vi "Matrix_Pow.vi"(10 "Exponent":dbl, 11 "input matrix":T1) -> (0 "Error":bool, 3 "output matrix":T1, 4 "ExponentNotRational":bool)   [LabVIEW 2019, in "Trajectory_Library.lvlib"]
doc: "Computes the matrix power using Eigen's solver. This method only works for square matrices, and will otherwise throw an MatrixDimensionException.\n \nInputs:\n - input matrix -- The input matrix\n - exponent -- The exponent.\n\nOutputs:\n - output matrix -- The exponential of A.\n - error -- If TRUE, an error occured.\n - ExponentNotRational -- TRUE if exponent is not a rational number."
uses:
  Trajectory_Library.lvlib
  <vilib>/Analysis/Matrix/Datatypes/RealMatrix.ctl
  <vilib>/Analysis/7linalg.llb/Real Matrix Power.vi
  <vilib>/Analysis/7linalg.llb/Real Matrix Exp.vi
  <vilib>/Analysis/7linalg.llb/Real Matrix Logarithm.vi
  <vilib>/Analysis/Matrix/Numeric/Complex/Complex To Cartesian - CM.vi
  <vilib>/Analysis/Matrix/Numeric/Multiply/Multiply - RM,R.vi
  <vilib>/Analysis/NI_AALBase.lvlib
  <vilib>/Analysis/Matrix/NI_Matrix.lvlib
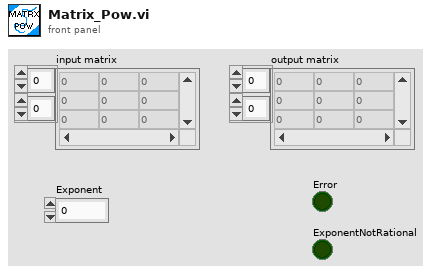
[diagram p1: front panel]
types:
  T1 = typedef "NI_Matrix.lvlib/RealMatrix.ctl" = dbl[][]
  T2 = typedef "NI_Matrix.lvlib/ComplexMatrix.ctl" = cdb[][]
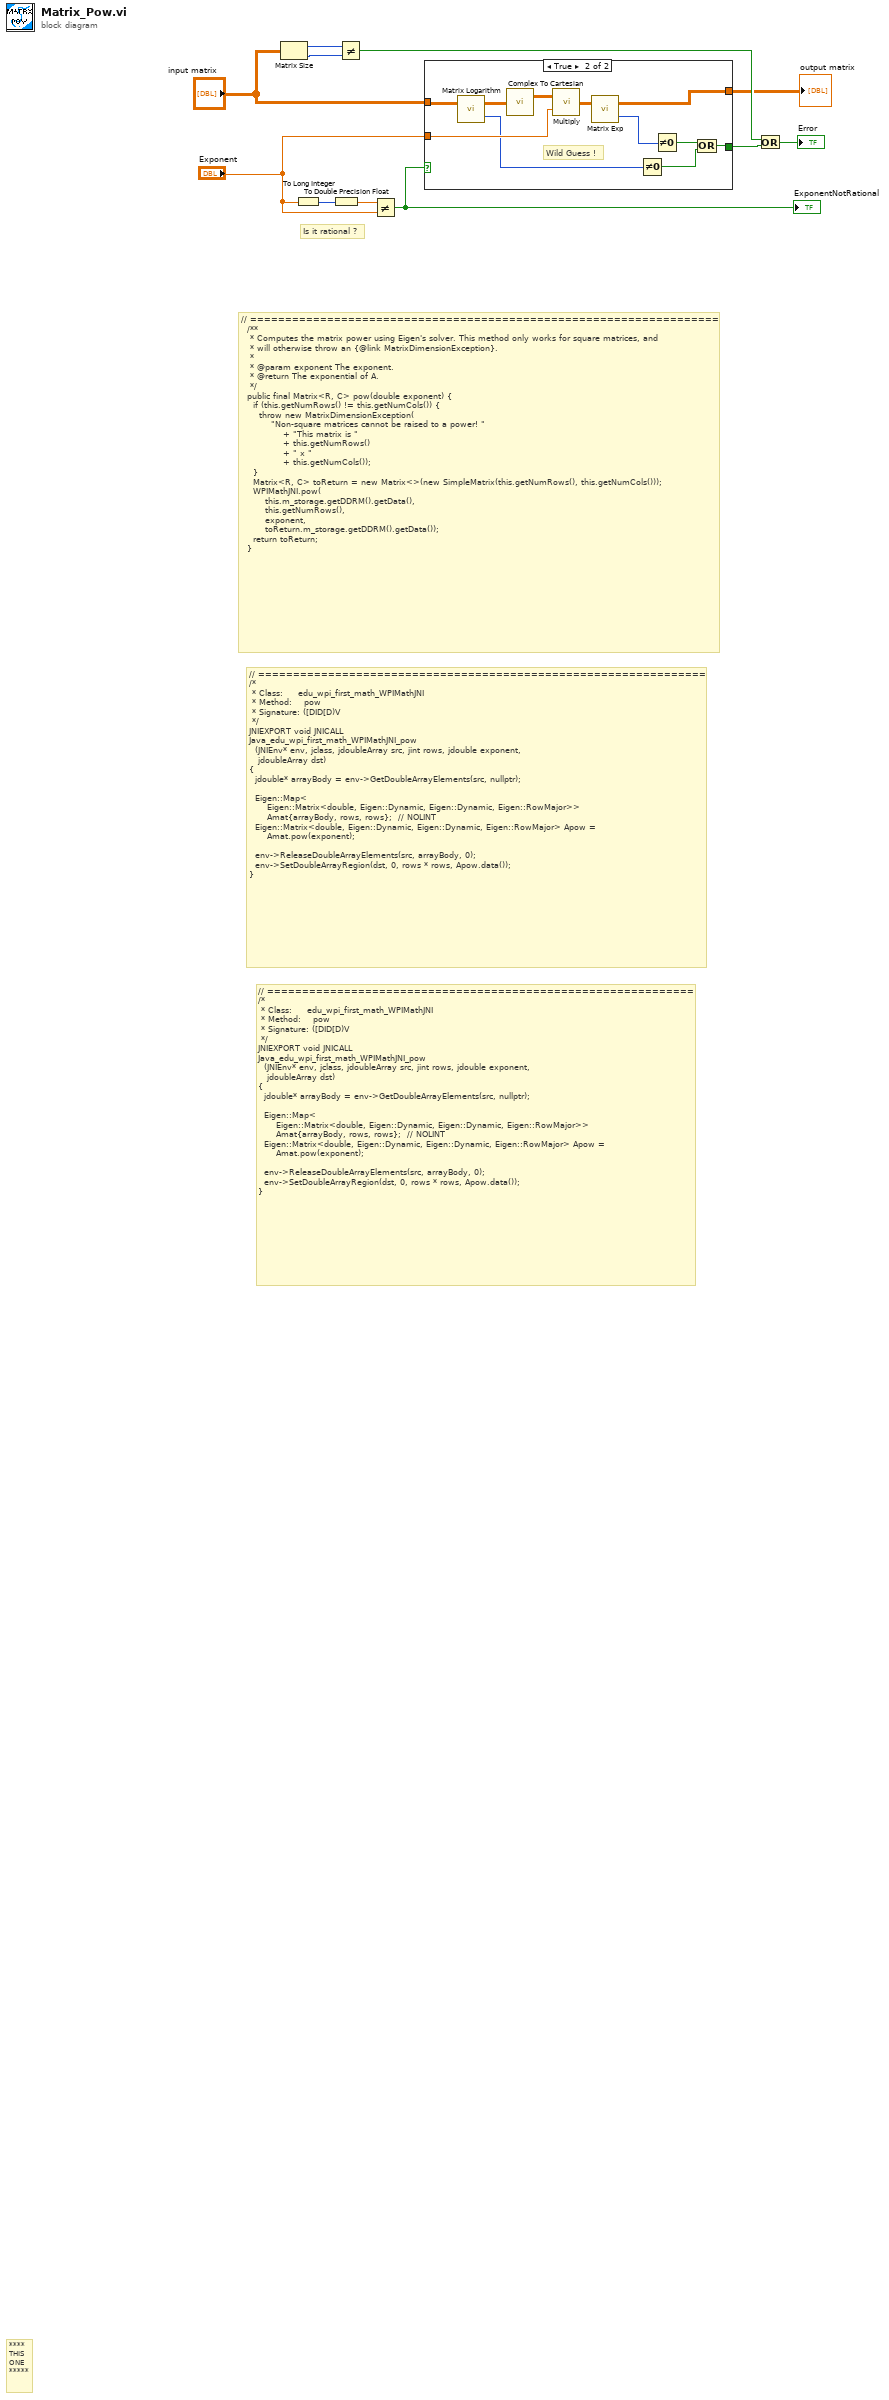
[diagram p0: block diagram]
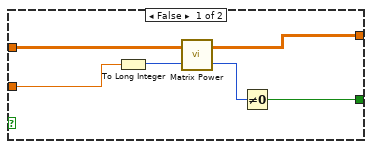
[diagram p2: hidden frame]
diagram:
  # "Is it rational ?"
  # "// =============================================================\n/*\n * Class:     edu_wpi_first_math_WPIMathJNI\n * Method:    pow\n * Signature: ([DID[D)V\n */\nJNIEXPORT void JNICALL\nJava_edu_wpi_first_math_WPIMathJNI_pow\n  (JNIEnv* env, jclass, jdoubleArray src, jint rows, jdouble exponent,\n   jdoubleArray dst)\n{\n  jdouble* arrayBody = env->GetDoubleArrayElements(src, nullptr);\n\n  Eigen::Map<\n      Eigen::Matrix<double, Eigen::Dynamic, Eigen::Dynamic, Eigen::RowMajor>>\n      Amat{arrayBody, rows, rows};  // NOLINT\n  Eigen::Matrix<double, Eigen::Dynamic, Eigen::Dynamic, Eigen::RowMajor> Apow =\n      Amat.pow(exponent);\n\n  env->ReleaseDoubleArrayElements(src, arrayBody, 0);\n  env->SetDoubleArrayRegion(dst, 0, rows * rows, Apow.data());\n}"
  # "// ================================================================\n/*\n * Class:     edu_wpi_first_math_WPIMathJNI\n * Method:    pow\n * Signature: ([DID[D)V\n */\nJNIEXPORT void JNICALL\nJava_edu_wpi_first_math_WPIMathJNI_pow\n  (JNIEnv* env, jclass, jdoubleArray src, jint rows, jdouble exponent,\n   jdoubleArray dst)\n{\n  jdouble* arrayBody = env->GetDoubleArrayElements(src, nullptr);\n\n  Eigen::Map<\n      Eigen::Matrix<double, Eigen::Dynamic, Eigen::Dynamic, Eigen::RowMajor>>\n      Amat{arrayBody, rows, rows};  // NOLINT\n  Eigen::Matrix<double, Eigen::Dynamic, Eigen::Dynamic, Eigen::RowMajor> Apow =\n      Amat.pow(exponent);\n\n  env->ReleaseDoubleArrayElements(src, arrayBody, 0);\n  env->SetDoubleArrayRegion(dst, 0, rows * rows, Apow.data());\n}"
  # "// ===================================================================\n  /**\n   * Computes the matrix power using Eigen's solver. This method only works for square matrices, and\n   * will otherwise throw an {@link MatrixDimensionException}.\n   *\n   * @param exponent The exponent.\n   * @return The exponential of A.\n   */\n  public final Matrix<R, C> pow(double exponent) {\n    if (this.getNumRows() != this.getNumCols()) {\n      throw new MatrixDimensionException(\n          \"Non-square matrices cannot be raised to a power! \"\n              + \"This matrix is \"\n              + this.getNumRows()\n              + \" x \"\n              + this.getNumCols());\n    }\n    Matrix<R, C> toReturn = new Matrix<>(new SimpleMatrix(this.getNumRows(), this.getNumCols()));\n    WPIMathJNI.pow(\n        this.m_storage.getDDRM().getData(),\n        this.getNumRows(),\n        exponent,\n        toReturn.m_storage.getDDRM().getData());\n    return toReturn;\n  }"
  # "****\nTHIS\nONE\n*****"
  n1 = Matrix Size(0:"input matrix") -> (1:w11:i32, 2:w10:i32)
  n2 = To Long Integer(number="Exponent") -> (32bit integer=w7:i32)
  n3 = To Double Precision Float(number=w7) -> (double precision float=w6:dbl)
  n4 = Not Equal?(x=w11, y=w10) -> (x != y?=w8:bool)
  n5 = Not Equal?(x=w6, y="Exponent") -> (x != y?=w5:bool)
  "ExponentNotRational" <- w5
  n6 = case shown="True" w5 {
    tunnel: "input matrix" -> [w17 w28]
    tunnel: "Exponent" -> [w12 w27]
    tunnel: [w15 w26] -> w2
    tunnel: [w14 w18] -> w1
    frame False {
      n7 = To Long Integer(number=w12) -> (32bit integer=w13:i32)
      n8 = call-poly <vilib>:"Matrix Power.vi"("n"=w13, "Input Matrix"=w17) -> ("error"=w16:i32, "Matrix Power"=w14:T1)
      n9 = Not Equal To 0?(x=w16) -> (x != 0?=w15:bool)
    }
    frame True {
      # "Wild Guess !"
      n10 = call-poly <vilib>:"Matrix Logarithm.vi"("Input Matrix"=w28) -> ("error"=w24:i32, "Matrix Logarithm"=w22:T2)  [unwired: 1 in]
      n11 = call-poly <vilib>:"Complex To Cartesian.vi"("Complex Matrix R + Ii"=w22) -> ("Real Matrix R"=w21:T1)  [unwired: 1 out]
      n12 = call-poly <vilib>:"Multiply.vi"("Real Scalar c"=w27, "Real Matrix A"=w21) -> ("A * c"=w20:T1)
      n13 = call-poly <vilib>:"Matrix Exp.vi"("Input Matrix"=w20) -> ("error"=w19:i32, "Matrix Exp"=w18:T1)  [unwired: 1 in]
      n14 = Not Equal To 0?(x=w24) -> (x != 0?=w23:bool)
      n15 = Not Equal To 0?(x=w19) -> (x != 0?=w25:bool)
      n16 = Or(x=w25, y=w23) -> (x .or. y?=w26:bool)
    }
  }
  "output matrix" <- w1
  n17 = Or(x=w8, y=w2) -> (x .or. y?=→"Error":bool)
